vi "Data Readers and Writers NEW.vi"(8 "error in (no error)":errorcluster, 9 "Owning VI Details":T1, 10 "Full Element Name":string[](array[string]), 11 "synchronization":refnum<class "synchronization.lvclass">) -> (0 "error out":errorcluster)   [LabVIEW 2020]
uses:
  synchronization/synchronization.lvclass
  synchronization/synchronization.lvclass/synchronization.ctl
  JKI State Machine API/source/JKI SM/JKI SM.lvclass/JKI SM.ctl
  f42ed989-8671-4cdf-8706-bf1e8fb35ac6.vi
  <vilib>/Utility/error.llb/Clear Errors.vi
  <userlib>/_OpenG.lib/error/error.llb/Filter Error Codes (Array)__ogtk.vi
  <vilib>/regexp/Match Regular Expression.xnode
  <userlib>/_OpenG.lib/comparison/comparison.llb/openg_comparison__ogtk.lvlib
  JKI State Machine API/source/JKI SM/JKI SM.lvclass
  <userlib>/_OpenG.lib/error/error.llb/openg_error.lvlib
  <userlib>/_OpenG.lib/string/string.llb/openg_string.lvlib
  <userlib>/_OpenG.lib/comparison/comparison.llb/I32 Changed__ogtk.vi
  <userlib>/_OpenG.lib/comparison/comparison.llb/Boolean Changed__ogtk.vi
panel:
  in  "Listbox":i32(listbox)
  in  "OK":bool
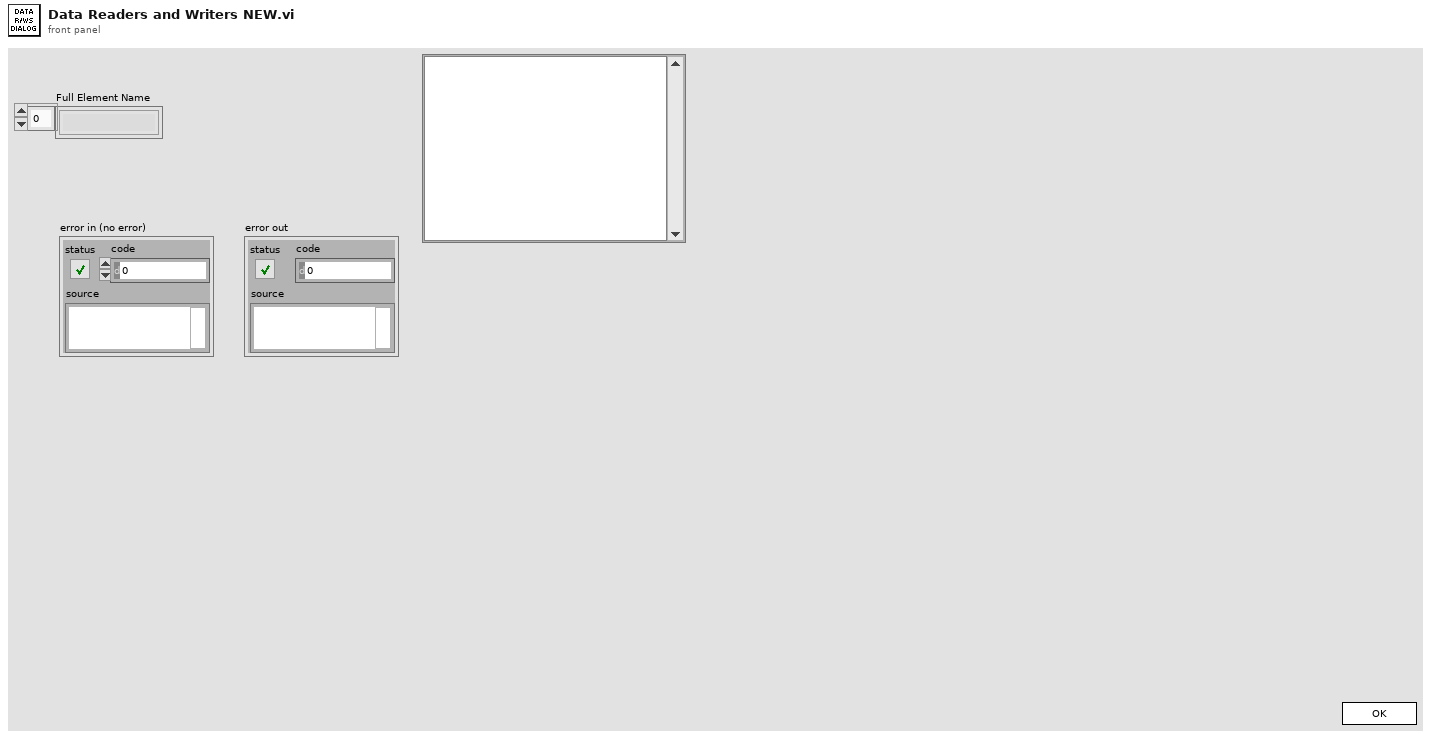
[diagram p1: front panel]
types:
  T1 = cluster{"App.ContextName":string, "VI.Name":string, "Object UID":i32}
  T2 = enum32{"Invalid", "Standard", "Closed", "Hidden", "Minimized", "Maximized"}
  T3 = enum32{"invalid app kind", "Development System", "Run Time System", "Student Edition", "Embedded LabVIEW", "Evaluation", "Custom"}
  T4 = enum32{"Invalid", "Default", "Floating", "Floating/Auto-Hide", "Modal"}
  T5 = cluster{"Core":cluster{"Current VI Reference":refnum<vi>, "Close Panel on Exit?":bool}, "Your Boolean data":bool, "Your string data":string, "Full Element Name":string[], "JKI SM out":refnum<class "JKI SM.lvclass">, "Callers":cluster{"(Un)Bundler":refnum<vi>, "Structure":string, "Frame Name":string}[], "GObject":refnum<vi>}
  T6 = cluster{"(Un)Bundler":refnum<vi>, "Structure":string, "Frame Name":string}[]
  T7 = cluster{"GObject":refnum<vi>, "Structure":string, "Frame Name":string}
  T8 = cluster{"(Un)Bundler":refnum<vi>, "Structure":string, "Frame Name":string}
  T9 = typedef "LVPoint32TypeDef.ctl" = cluster{"Horizontal":i32, "Vertical":i32}
  T10 = cluster{"Shift":bool, "Ctrl":bool, "Alt":bool, "Cmd":bool, "Opt":bool}
  T11 = cluster{"StringConstant":refnum<vi>, "Structure":string, "Frame Name":string, "State Call":string, "UID":dbl}[]
  T12 = cluster{"Current VI Reference":refnum<vi>, "Close Panel on Exit?":bool}
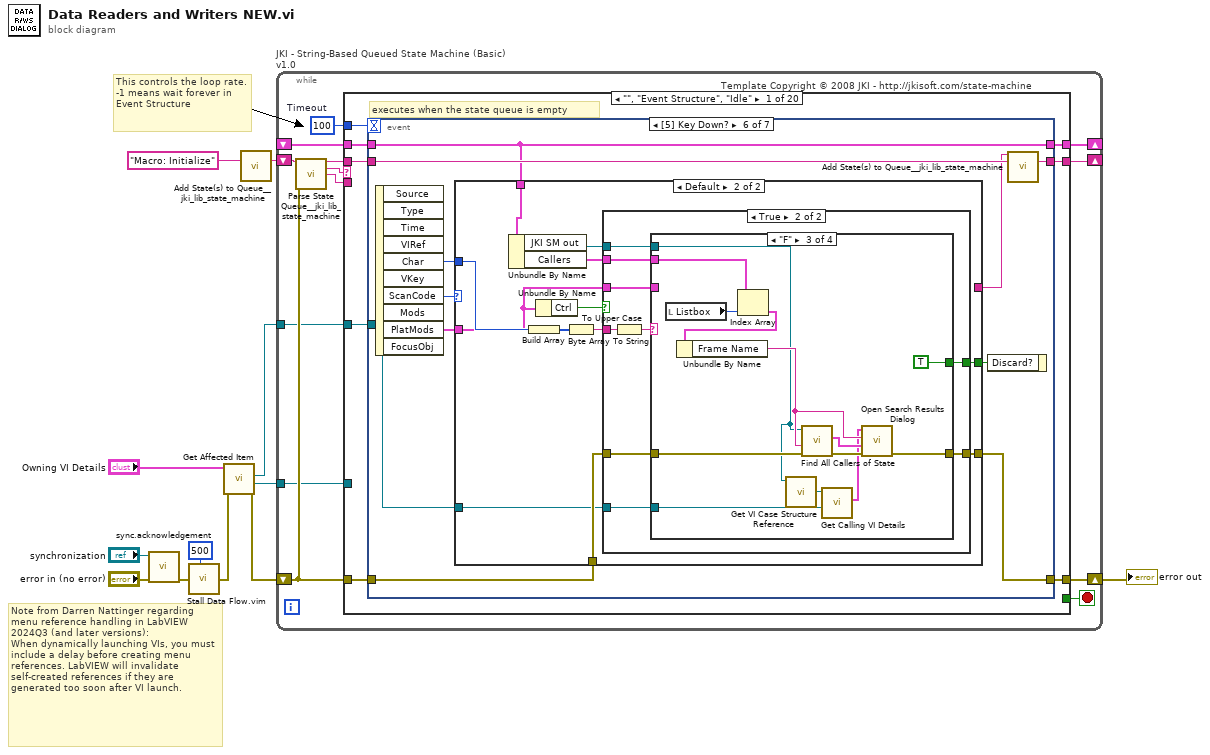
[diagram p0: block diagram]
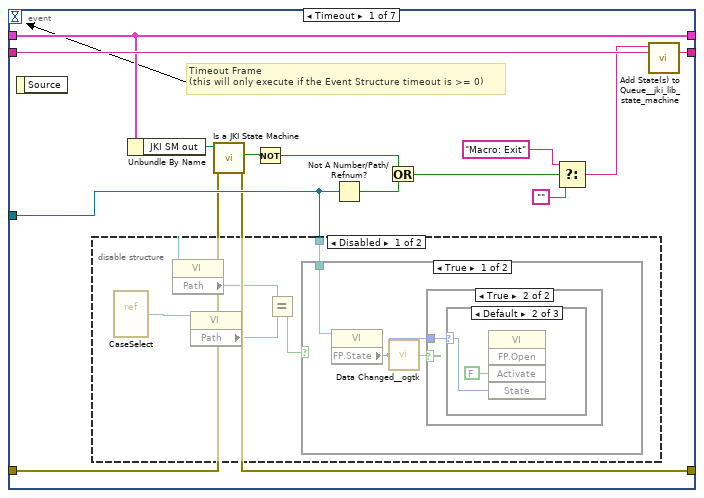
[diagram p2: hidden frame]
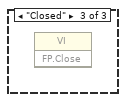
[diagram p5: hidden frame]
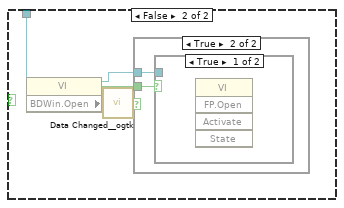
[diagram p6: hidden frame]
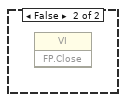
[diagram p8: hidden frame]
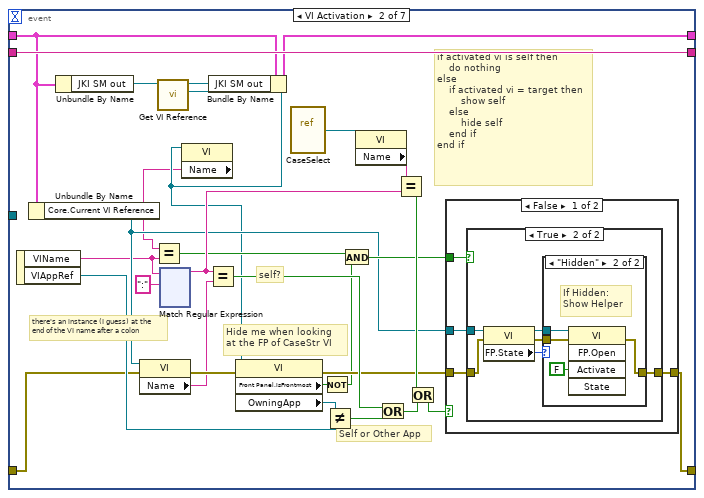
[diagram p10: hidden frame]
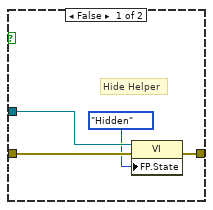
[diagram p11: hidden frame]
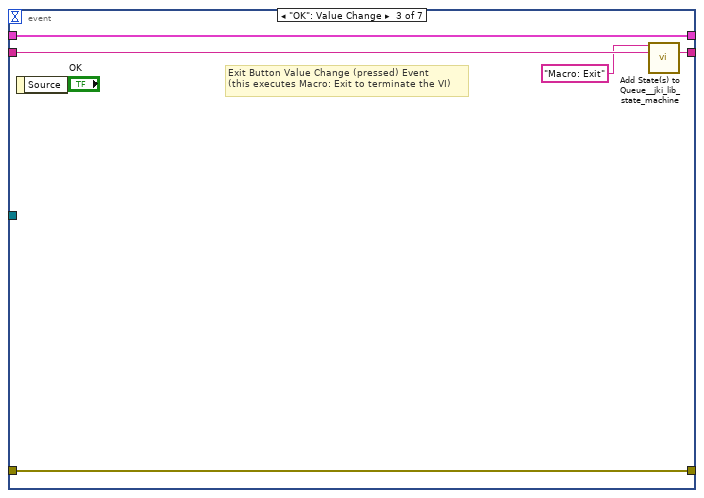
[diagram p14: hidden frame]
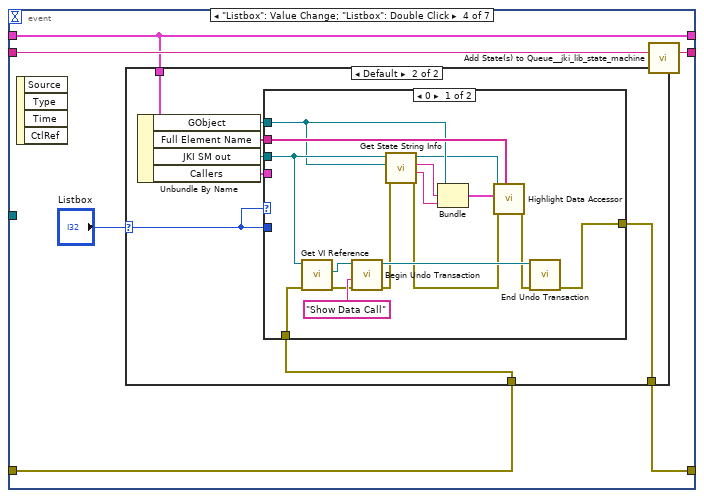
[diagram p15: hidden frame]
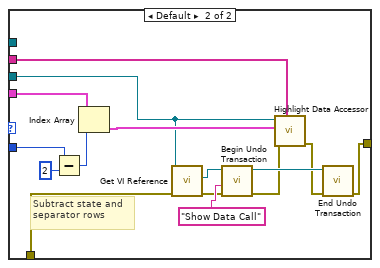
[diagram p17: hidden frame]
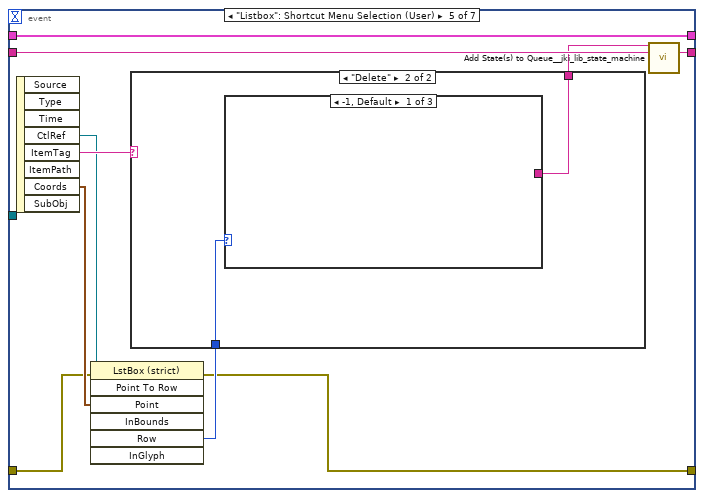
[diagram p18: hidden frame]
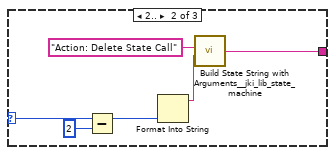
[diagram p20: hidden frame]
diagram:
  # "Note from Darren Nattinger regarding menu reference handling in LabVIEW 2024Q3 (and later versions):\nWhen dynamically launching VIs, you must include a delay before creating menu references. LabVIEW will invalidate self-created references if they are generated too soon after VI launch."
  # "This controls the loop rate. -1 means wait forever in Event Structure"
  n1 = call "sync.acknowledgement.vi"("error in (no error)"="error in (no error)", "synchronization"="synchronization") -> ("error out"=w2:errorcluster)  [unwired: 9 in]
  n2 = call "Stall Data Flow.vim"("value in"=w2, "milliseconds to wait"=u32 500) -> ("value out"=w5:errorcluster)  [unwired: 1 out]
  n3 = call "Get Affected Item.vi"("error in (no error)"=w5, "Owning VI Details"="Owning VI Details") -> ("error out"=w6:errorcluster, "GObject"=w9:refnum<vi>, "Owning VI"=w8:refnum<vi>)  [unwired: 6 in, 1 out]
  n4 = call <vilib>:"Add State(s) to Queue__jki_lib_state_machine.vi"("State(s) in (\"\")"="Macro: Initialize") -> ("States Out"=w12:string)  [unwired: 14 in]
  n5 = while "JKI - String-Based Queued State Machine (Basic) v1.0" {
    shift-right: [w18] -> _
    shift-left: _ -> [w17]
    shift-right: [w21] -> w10
    shift-left: w6 -> [w15]
    shift-right: [w20] -> _
    shift-left: w12 -> [w22]
    tunnel: w8 -> [w14]
    tunnel: w9 -> [w13]
    stop <- w19 stop-if-true
    w16 = 100  # Timeout
    # "Template Copyright © 2008 JKI - http://jkisoft.com/state-machine"
    n6 = call <vilib>:"Parse State Queue__jki_lib_state_machine.vi"("State Queue"=w22, "Error In (no error)"=w15) -> ("Remaining States"=w24:string, "Current State"=w25:string, "Arguments"=w23:string)  [unwired: 11 in]
    n7 = case shown="\"\", \"Event Structure\", \"Idle\"" w25 {
      selector: w25 -> [_ _ w388 _ _ _ _ _ _ _ _ _ _ _ _ _ _ _ _ _]
      tunnel: w24 -> [w33 w387 w392 w412 w423 w428 w432 w444 w458 w464 w485 w503 w523 w534 w563 w568 w578 w582 w599 w643]
      tunnel: w23 -> [_ _ _ _ _ _ _ _ _ _ _ _ w518 w528 _ _ _ _ _ _]
      tunnel: w17 -> [w31 w384 w390 w404 w420 w426 w429 _ w455 w461 w483 w497 w521 w530 w560 w566 w575 w579 w595 w641]
      tunnel: [w30 w385 w394 w399 errorcluster {"status"=FALSE, "code"=0, "source"=""} ("error out") w425 w430 w433 w451 w462 w465 w494 w519 w531 w561 w564 w576 w580 w587 w626] -> w21
      tunnel: w15 -> [w29 w385 w393 w400 w418 w425 w430 w434 w446 w462 w465 w495 w520 w532 w561 w564 w576 w580 w596 w625]
      tunnel: [w32 w386 w391 w411 w422 w427 w431 w443 w457 w463 w484 w502 w522 w533 w562 w567 w577 w581 w598 w642] -> w20
      tunnel: [_ _ _ _ _ TRUE _ _ _ _ _ _ _ _ _ _ _ _ _ _] -> w19
      tunnel: [w28 w384 w390 w410 w420 w426 w429 w442 w455 w461 w483 w497 w521 w530 w560 w566 w575 w579 w584 w640] -> w18
      tunnel: w16 -> [w27 _ _ _ _ _ _ _ _ _ _ _ _ _ _ _ _ _ _ _]
      tunnel: w14 -> [w26 _ _ _ _ _ _ _ _ _ _ _ _ _ _ _ _ _ _ _]
      tunnel: w13 -> [_ _ _ _ _ _ _ w436 _ _ _ _ _ _ _ _ _ _ _ _]
      frame "", "Event Structure", "Idle" {
        # "executes when the state queue is empty"
        n8 = event shown="[5] Key Down?" {
          selector: _ -> [_ _ _ _ _ _ _]
          dyn-events: _ -> [_ _ _ _ _ _ _]
          timeout: w27 -> [_ _ _ _ _ _ _]
          tunnel: w33 -> [w47 w93 w229 w235 w285 w306 w383]
          tunnel: [w46 w93 w228 w234 w284 w305 w382] -> w32
          tunnel: w31 -> [w41 w67 w226 w233 w277 w304 w380]
          tunnel: [w36 w68 w227 w231 w276 w299 w381] -> w30
          tunnel: w29 -> [w37 w69 w227 w232 w279 w300 w381]
          tunnel: [w41 w66 w226 w233 w277 w304 w380] -> w28
          tunnel: w26 -> [w42 _ _ _ _ w296 _]
          event Timeout {
            # "Timeout Frame\n(this will only execute if the Event Structure timeout is >= 0)"
            n9 = event-data() -> ()  [unwired: 1 in, 1 out]
            n10 = disable-structure shown="Disabled" {
              disable-tunnel: w42 -> [w48 _]
              frame Disabled {
                n11 = vi-ref "CaseSelect.vi"() -> (w50:refnum<vi>)
                n12 = property class="VI"(reference=w48) -> ("Path"=w49:path)  [unwired: 1 in, 2 out]
                n13 = property class="VI"(reference=w50) -> ("Path"=w52:path)  [unwired: 1 in, 2 out]
                n14 = Equal?(x=w49, y=w52) -> (x = y?=w51:bool)
                n15 = case shown="True" w51 {
                  tunnel: w48 -> [w53 w60]
                  frame True {
                    n16 = property class="VI"(reference=w53) -> ("FP.State"=w54:T2)  [unwired: 1 in, 2 out]
                    n17 = call-poly <userlib>:"Data Changed__ogtk.vi"("I32"=w54) -> ("Changed"=w55:bool)
                    n18 = case shown="True" w55 {
                      tunnel: w54 -> [_ w56]
                      frame False {
                      }
                      frame True {
                        n19 = case shown="Default" w56 {
                          selector: w56 -> [_ w57 _]
                          frame "Invalid" {
                          }
                          frame Default {
                            n20 = invoke class="VI" method="FP.Open"("Activate"=FALSE ("Activate?"), "State"=w57) -> ()  [unwired: 3 in, 5 out]
                          }
                          frame "Closed" {
                            n21 = invoke class="VI" method="FP.Close"() -> ()  [unwired: 3 in, 3 out]
                          }
                        }
                      }
                    }
                  }
                  frame False {
                    n22 = property class="VI"(reference=w60) -> (reference out=w59:refnum<vi>, "BDWin.Open"=w61:bool)  [unwired: 1 in, 1 out]
                    n23 = call-poly <userlib>:"Data Changed__ogtk.vi"("Boolean"=w61) -> ("Changed"=w62:bool)
                    n24 = case shown="True" w62 {
                      tunnel: w61 -> [_ w64]
                      tunnel: w59 -> [_ w63]
                      frame False {
                      }
                      frame True {
                        n25 = case shown="True" w64 {
                          tunnel: w63 -> [_ _]
                          frame True {
                            n26 = invoke class="VI" method="FP.Open"() -> ()  [unwired: 5 in, 5 out]
                          }
                          frame False {
                            n27 = invoke class="VI" method="FP.Close"() -> ()  [unwired: 3 in, 3 out]
                          }
                        }
                      }
                    }
                  }
                }
              }
              frame Enabled {
              }
            }
            n28 = Unbundle By Name(w41) -> ("JKI SM out"=w40:refnum<class "JKI SM.lvclass">)
            n29 = call "Is a JKI State Machine.vi"("error in (no error)"=w37, "JKI SM in"=w40) -> ("error out"=w36:errorcluster, "Is a JKI State Machine"=w39:bool)  [unwired: 7 in, 1 out]
            n30 = Not(x=w39) -> (.not. x?=w38:bool)
            n31 = Not A Number/Path/Refnum?(number/path/refnum=w42) -> (NaN/Path/Refnum?=w35:bool)
            n32 = Or(x=w38, y=w35) -> (x .or. y?=w34:bool)
            n33 = Select(t="Macro: Exit", s=w34, f="") -> (s? t:f=w43:string)
            n34 = call <vilib>:"Add State(s) to Queue__jki_lib_state_machine.vi"("State(s) in Front (\"\")"=w43, "State(s) in (\"\")"=w47) -> ("States Out"=w46:string)  [unwired: 13 in]
          }
          event VI Activation {
            # "Self or Other App"
            # "self?"
            # "Hide me when looking\nat the FP of CaseStr VI"
            # "there's an instance (I guess) at the\nend of the VI name after a colon"
            # "if activated vi is self then\n    do nothing\nelse\n    if activated vi = target then\n        show self\n    else\n        hide self\n    end if\nend if"
            n35 = event-data() -> ("VIName"=w71:string, "VIAppRef"=w70:refnum<vi>)  [unwired: 1 in]
            n36 = Unbundle By Name(w67) -> ("Core.Current VI Reference"=w78:refnum<vi>)
            n37 = Unbundle By Name(w67) -> ("JKI SM out"=w74:refnum<class "JKI SM.lvclass">)
            n38 = property class="VI"(reference=w78, error in=w69) -> (error out=w82:errorcluster, "Name"=w77:string)  [unwired: 1 out]
            n39 = call "Get VI Reference.vi"("JKI SM in"=w74) -> ("VI"=w73:refnum<vi>, "JKI SM out"=w65:refnum<class "JKI SM.lvclass">)  [unwired: 8 in, 1 out]
            n40 = xnode "Match Regular Expression"("input string"=w71, "regular expression"=":") -> ("before match"=w89:string)  [unwired: 3 in, 5 out]
            n41 = property class="VI"(reference=w73) -> ("Name"=w72:string)  [unwired: 1 in, 2 out]
            n42 = Equal?(x=w72, y=w71) -> (x = y?=w75:bool)
            n43 = Equal?(x=w89, y=w77) -> (x = y?=w86:bool)
            n44 = Bundle By Name(cluster=w67, "JKI SM out"=w65) -> (w66:T5)
            n45 = property class="VI"(reference=w73, error in=w82) -> (error out=w81:errorcluster, "Front Panel.IsFrontmost"=w79:bool, "OwningApp"=w84:refnum<vi>)  [unwired: 1 out]
            n46 = vi-ref "CaseSelect.vi"() -> (w87:refnum<vi>)
            n47 = Not(x=w79) -> (.not. x?=w80:bool)
            n48 = Not Equal?(x=w84, y=w70) -> (x != y?=w85:bool)
            n49 = And(x=w75, y=w80) -> (x .and. y?=w83:bool)
            n50 = property class="VI"(reference=w87) -> ("Name"=w88:string)  [unwired: 1 in, 2 out]
            n51 = Or(x=w86, y=w85) -> (x .or. y?=w91:bool)
            n52 = Equal?(x=w88, y=w89) -> (x = y?=w90:bool)
            n53 = Or(x=w90, y=w91) -> (x .or. y?=w92:bool)
            n54 = case shown="False" w92 {
              tunnel: w81 -> [w97 w113]
              tunnel: [w95 w113] -> w68
              tunnel: w78 -> [w96 _]
              tunnel: w83 -> [w94 _]
              frame False {
                n55 = case shown="True" w94 {
                  tunnel: w97 -> [w101 w106]
                  tunnel: w96 -> [w100 w107]
                  tunnel: [w99 w104] -> w95
                  frame False {
                    # "Hide Helper"
                    n56 = property class="VI"(reference=w100, error in=w101, "FP.State"=T2."Hidden" ("Front Panel Window:State")) -> (error out=w99:errorcluster)  [unwired: 1 out]
                  }
                  frame True {
                    n57 = property class="VI"(reference=w107, error in=w106) -> (reference out=w103:refnum<vi>, error out=w102:errorcluster, "FP.State"=w105:T2)
                    n58 = case shown="\"Hidden\"" w105 {
                      tunnel: [w108 w112] -> w104
                      tunnel: w103 -> [_ w111]
                      tunnel: w102 -> [w108 w110]
                      frame Default {
                      }
                      frame "Hidden" {
                        # "If Hidden:\nShow Helper"
                        n59 = invoke class="VI" method="FP.Open"(reference=w111, error in=w110, "Activate"=FALSE ("Activate?")) -> (error out=w112:errorcluster)  [unwired: 2 in, 4 out]
                      }
                    }
                  }
                }
              }
              frame True {
              }
            }
          }
          event "OK": Value Change {
            # "Exit Button Value Change (pressed) Event\n(this executes Macro: Exit to terminate the VI)"
            n60 = event-data() -> ()  [unwired: 1 in, 1 out]
            n61 = call <vilib>:"Add State(s) to Queue__jki_lib_state_machine.vi"("State(s) in Front (\"\")"="Macro: Exit", "State(s) in (\"\")"=w229) -> ("States Out"=w228:string)  [unwired: 13 in]
          }
          event "Listbox": Value Change; "Listbox": Double Click {
            n62 = event-data() -> ()  [unwired: 1 in, 4 out]
            n63 = case shown="Default" "Listbox" {
              selector: "Listbox" -> [_ w238]
              tunnel: w233 -> [_ w244]
              tunnel: w232 -> [w236 w241]
              tunnel: [w236 w240] -> w231
              frame -1 {
              }
              frame Default {
                n64 = Unbundle By Name(w244) -> ("GObject"=w237:refnum<vi>, "Full Element Name"=w239:string[], "JKI SM out"=w242:refnum<class "JKI SM.lvclass">, "Callers"=w243:T6)
                n65 = case shown="0" w238 {
                  tunnel: w243 -> [_ w275]
                  tunnel: w242 -> [w258 w266]
                  tunnel: w241 -> [w259 w262]
                  tunnel: w238 -> [_ w271]
                  tunnel: [w257 w263] -> w240
                  tunnel: w239 -> [w260 w273]
                  tunnel: w237 -> [w256 _]
                  frame 0 {
                    n66 = call "Get VI Reference.vi"("error in (no error)"=w259, "JKI SM in"=w258) -> ("error out"=w254:errorcluster, "VI"=w253:refnum<vi>)  [unwired: 7 in, 1 out]
                    n67 = call "Begin Undo Transaction.vi"("error in (no error)"=w254, "Action"="Show Data Call", "VI in"=w253) -> ("error out"=w246:errorcluster, "VI out"=w252:refnum<vi>)  [unwired: 7 in]
                    n68 = call "Get State String Info.vi"("error in (no error)"=w246, "GObj Refnum in"=w256, "JKI SM in"=w258) -> ("error out"=w245:errorcluster, "Frame Name"=w249:string, "Structure"=w250:string, "JKI SM out"=w251:refnum<class "JKI SM.lvclass">)  [unwired: 5 in]
                    n69 = Bundle("GObject"=w256, "Structure"=w250, "Frame Name"=w249) -> (w248:T7)  [unwired: 1 in]
                    n70 = call "Highlight Data Accessor.vi"("Full Element Name"=w260, "error in (no error)"=w245, "Cluster"=w248, "JKI SM in"=w251) -> ("error out"=w247:errorcluster)  [unwired: 6 in, 1 out]
                    n71 = call "End Undo Transaction.vi"("error in (no error)"=w247, "VI in"=w252) -> ("error out"=w257:errorcluster)  [unwired: 8 in, 1 out]
                  }
                  frame Default {
                    # "Subtract state and separator rows"
                    n72 = Subtract(x=w271, y=2) -> (x-y=w270:i32)
                    n73 = Index Array(array=w275, index=w270) -> (element=w274:T8)
                    n74 = call "Get VI Reference.vi"("error in (no error)"=w262, "JKI SM in"=w266) -> ("error out"=w268:errorcluster, "VI"=w267:refnum<vi>)  [unwired: 7 in, 1 out]
                    n75 = call "Begin Undo Transaction.vi"("error in (no error)"=w268, "Action"="Show Data Call", "VI in"=w267) -> ("error out"=w261:errorcluster, "VI out"=w265:refnum<vi>)  [unwired: 7 in]
                    n76 = call "Highlight Data Accessor.vi"("Full Element Name"=w273, "error in (no error)"=w261, "Cluster"=w274, "JKI SM in"=w266) -> ("error out"=w264:errorcluster)  [unwired: 6 in, 1 out]
                    n77 = call "End Undo Transaction.vi"("error in (no error)"=w264, "VI in"=w265) -> ("error out"=w263:errorcluster)  [unwired: 8 in, 1 out]
                  }
                }
              }
            }
            n78 = call <vilib>:"Add State(s) to Queue__jki_lib_state_machine.vi"("State(s) in (\"\")"=w235) -> ("States Out"=w234:string)  [unwired: 14 in]
          }
          event "Listbox": Shortcut Menu Selection (User) {
            n79 = event-data() -> ("CtlRef"=w282:refnum<vi>, "ItemTag"=w283:string, "Coords"=w281:T9)  [unwired: 1 in, 5 out]
            n80 = invoke class="LstBox (strict)" method="Point To Row"(reference=w282, error in=w279, "Point"=w281) -> (error out=w276:errorcluster, "Row"=w280:i32)  [unwired: 4 in, 5 out]
            n81 = case shown="\"Delete\"" w283 {
              tunnel: w280 -> [_ w287]
              tunnel: [_ w286] -> w278
              frame Default {
              }
              frame "Delete" {
                n82 = case shown="-1, Default" w287 {
                  selector: w287 -> [_ w290 _]
                  tunnel: [_ w291 w294] -> w286
                  frame -1, Default {
                  }
                  frame 2.. {
                    n83 = Subtract(x=w290, y=2) -> (x-y=w289:i32)
                    n84 = Format Into String(w289) -> (resulting string=w292:string)  [unwired: 3 in, 1 out]
                    n85 = call <vilib>:"Build State String with Arguments__jki_lib_state_machine.vi"("Arguments (\"\")"=w292, "State"="Action: Delete State Call") -> ("State with Arguments"=w291:string)  [unwired: 4 in]
                  }
                  frame 0 {
                    n86 = call <vilib>:"Build State String with Arguments__jki_lib_state_machine.vi"("State"="Action: Delete State") -> ("State with Arguments"=w294:string)  [unwired: 5 in]
                  }
                }
              }
            }
            n87 = call <vilib>:"Add State(s) to Queue__jki_lib_state_machine.vi"("State(s) in Front (\"\")"=w278, "State(s) in (\"\")"=w285) -> ("States Out"=w284:string)  [unwired: 13 in]
          }
          event Key Down? {
            n88 = event-data() -> ("Char"=w303:i16, "ScanCode"=w298:i16, "PlatMods"=w302:T10)  [unwired: 1 in, 7 out]
            n89 = case shown="Default" w298 {
              tunnel: w304 -> [_ w325]
              tunnel: w303 -> [_ w323]
              tunnel: w302 -> [_ w320]
              tunnel: [_ w318] -> w301
              tunnel: w300 -> [w308 w316]
              tunnel: [w308 w315] -> w299
              tunnel: [w307 _] -> w297
              tunnel: w296 -> [_ w314]
              frame 83 {
                n90 = local read "Listbox"() -> (w309:i32)
                n91 = case shown="Default" w309 {
                  selector: w309 -> [_ w310]
                  tunnel: [_ w311] -> w307
                  frame -1 {
                  }
                  frame Default {
                    n92 = Format Into String(w310) -> (resulting string=w312:string)  [unwired: 3 in, 1 out]
                    n93 = call <vilib>:"Build State String with Arguments__jki_lib_state_machine.vi"("Arguments (\"\")"=w312, "State"="Action: Delete State Call") -> ("State with Arguments"=w311:string)  [unwired: 4 in]
                  }
                }
              }
              frame Default {
                n94 = Unbundle By Name(w325) -> ("JKI SM out"=w317:refnum<class "JKI SM.lvclass">, "Callers"=w324:T6)
                n95 = Build Array(w323) -> (w322:i16[])
                n96 = Unbundle By Name(w320) -> ("Ctrl"=w319:bool)
                n97 = Byte Array To String(unsigned byte array=w322) -> (string=w321:string)
                n98 = case shown="True" w319 {
                  tunnel: w324 -> [_ w335]
                  tunnel: w321 -> [_ w334]
                  tunnel: w320 -> [_ w333]
                  tunnel: [_ w332] -> w318
                  tunnel: w317 -> [_ w330]
                  tunnel: [w326 w329] -> w315
                  tunnel: w316 -> [w326 w328]
                  tunnel: w314 -> [_ w327]
                  frame False {
                  }
                  frame True {
                    n99 = To Upper Case(1:w334) -> (0:w331:string)
                    n100 = case shown="\"F\"" w331 {
                      tunnel: w335 -> [_ w350 w361 _]
                      tunnel: w333 -> [_ w345 _ w370]
                      tunnel: [_ TRUE TRUE TRUE] -> w332
                      tunnel: w330 -> [_ _ w354 w367]
                      tunnel: [w336 w343 w355 w364] -> w329
                      tunnel: w328 -> [w336 w343 w356 w368]
                      tunnel: w327 -> [_ _ w351 _]
                      frame Default {
                      }
                      frame "G" {
                        w338 = 2 ("y")
                        n101 = local read "Listbox"() -> (w340:i32)
                        n102 = Unbundle By Name(w345) -> ("Shift"=w346:bool)
                        n103 = Array Size(array=w350) -> (size(s)=w337:i32)
                        n104 = Subtract(x=w340, y=w338) -> (x-y=w339:i32)
                        n105 = Decrement(x=w339) -> (x-1=w348:i32)
                        n106 = Increment(x=w339) -> (x+1=w349:i32)
                        n107 = Select(t=w348, s=w346, f=w349) -> (s? t:f=w347:i32)
                        n108 = Quotient & Remainder(x=w347, y=w337) -> (x-y*floor(x/y)=w342:i32)  [unwired: 1 out]
                        n109 = Add(x=w342, y=w338) -> (x+y=w341:i32)
                        n110 = property on="Listbox" class="LstBox (strict)"("Val(Sgnl)"=w341) -> ()  [unwired: 2 in, 2 out]
                      }
                      frame "F" {
                        n111 = local read "Listbox"() -> (w362:i32)
                        n112 = Index Array(array=w361, index=w362) -> (element=w360:T8)
                        n113 = Unbundle By Name(w360) -> ("Frame Name"=w357:string)
                        n114 = call "Get VI Case Structure Reference.vi"("JKI SM in"=w354) -> ("Case Structure ref"=w353:refnum<vi>)  [unwired: 8 in, 2 out]
                        n115 = call "Find All Callers of State.vi"("error in (no error)"=w356, "State Name"=w357, "JKI SM in"=w354) -> ("error out"=w358:errorcluster, "Callers"=w359:T11)  [unwired: 6 in, 1 out]
                        n116 = call "Get Calling VI Details.vi"("User VI Ref"=w351, "Affected Items"=w353) -> ("Calling VI Details"=w352:T1)  [unwired: 9 in]
                        n117 = call "Open Search Results Dialog.vi"("error in (no error)"=w358, "Callers"=w359, "State"=w357, "Calling VI Details"=w352) -> ("error out"=w355:errorcluster)  [unwired: 7 in]
                      }
                      frame "Z" {
                        # "Override Ctrl+Z and Ctrl+Shift+Z\n(Handle them here and target the user's VI)"
                        n118 = call "Get VI Reference.vi"("error in (no error)"=w368, "JKI SM in"=w367) -> ("error out"=w365:errorcluster, "VI"=w366:refnum<vi>)  [unwired: 7 in, 1 out]
                        n119 = Unbundle By Name(w370) -> ("Shift"=w369:bool)
                        n120 = case shown="False" w369 {
                          tunnel: w366 -> [w374 w377]
                          tunnel: w365 -> [w372 w376]
                          tunnel: [w373 w375] -> w364
                          frame False {
                            n121 = invoke class="VI" method="Transaction.Undo"(reference=w374, error in=w372) -> (error out=w373:errorcluster)  [unwired: 1 in, 2 out]
                          }
                          frame True {
                            n122 = invoke class="VI" method="Transaction.Redo"(reference=w377, error in=w376) -> (error out=w375:errorcluster)  [unwired: 1 in, 2 out]
                          }
                        }
                      }
                    }
                  }
                }
              }
            }
            n123 = event-data("Discard?"=w301) -> ()  [unwired: 1 in, 1 out]
            n124 = call <vilib>:"Add State(s) to Queue__jki_lib_state_machine.vi"("State(s) in Front (\"\")"=w297, "State(s) in (\"\")"=w306) -> ("States Out"=w305:string)  [unwired: 13 in]
          }
          event Panel Close? {
            # "Discard the event because we'll close the front panel ourselves in Macro: Exit"
            # "Close Panel button (pressed) Event\n(this executes Macro: Exit to terminate the VI)"
            n125 = event-data() -> ()  [unwired: 1 in, 1 out]
            n126 = event-data("Discard?"=TRUE) -> ()  [unwired: 1 in, 1 out]
            n127 = call <vilib>:"Add State(s) to Queue__jki_lib_state_machine.vi"("State(s) in Front (\"\")"="Macro: Exit", "State(s) in (\"\")"=w383) -> ("States Out"=w382:string)  [unwired: 13 in]
          }
        }
      }
      frame "---------- Core ----------" {
        # "Do not put any code in this frame.\n(it is a separator no-op)"
        n128 = call <vilib>:"Add State(s) to Queue__jki_lib_state_machine.vi"("State(s) in (\"\")"=w387) -> ("States Out"=w386:string)  [unwired: 14 in]
      }
      frame Default {
        w397 = 42 items=["No error", "Argument error", "Memory is full", "Out of zone", "End of file", "File already open", "Generic file I/O error", "File not found", "File permission error", "Disk is full", "Duplicate path", "Too many files open", "System feature not enabled", "Resource file not found", "Cannot add resource", "Resource not found", "Image not found", "Image memory error", "Pen does not exist", "Config type invalid", "Config token not found", "Config parse error", "Config memory error", "Bad external code format", "Bad external code offset", "External code not present", "Null window", "Destroy window error", "Null menu", "Print aborted", "Bad print record", "Print driver error", "Windows error during printing", "Memory error during printing", "Print dialog error", "Generic print error", "Invalid device refnum", "Device not found", "Device parameter error", "Device unit error", "Cannot open device", "Device call aborted", "Generic error", "Cancelled by user", "Object ID too low", "Object ID too high", "Object not in heap", "Unknown heap", "Unknown object (invalid DefProc)", "Unknown object (DefProc not in table)", "Message out of range", "Invalid (null) method", "Unknown message", "Manager call not supported", "Bad address", "Network operation in progress", "Network operation timed out", "Connection is busy", "Network attribute not supported", "Network error", "Address in use", "System out of memory", "Connection aborted", "Connection refused", "Not connected", "Already connected", "Connection closed", "Initialization error (interapplication manager)", "Bad occurrence", "Wait on unbound occurrence handler", "Occurrence queue overflow", "Datalog type conflict", "Unused", "Unrecognized type (interapplication manager)", "Memory corrupt", "Failed to make temporary DLL", "Old CIN version", "Drag socket not found", "Failed to load drop-object", "Failed to register OLE object", "Failed to release OLE object", "Format specifier type mismatch", "Unknown format specifier", "Too few format specifiers", "Too many format specifiers", "Scan failed", "Newer CIN version", "Error converting to variant", "Runtime menu error", "Password tampered", "Variant attribute not found", "Incompatible variant data type", "Event data is not available", "Event Store is not present", "Occurrence is not found", "Event Queue is not created", "Event info is not available", "Refnum passed is NULL", "Error retrieving Class GUID", "Error retrieving CoClass GUID", "Error retrieving TypeLib GUID.", "Bad built application magic bytes.", "Specific driver is different from the specific driver associated with the Logical Name.", "There is no session opened to the class driver.", "Max Error", "MAX - Error with config objects", "MAX - Error loading configuration", "MAX - Group not supported"]
        # "Current State"
        # "Do not delete, rename, or modify this frame.\n(this is used to capture unhandled states and typos)"
        # "Handle mistyped state name (developer tool)"
        n129 = Format Into String(format string="Software Exception: Unhandled State \"%s\"." ("message"), error in=w393, w388) -> (resulting string=w396:string, error out=w395:errorcluster)  [unwired: 1 in]
        n130 = call <vilib>:"Error Cluster From Error Code.vi"("show call chain? (False)"=TRUE, "error in (no error)"=w395, "error message (\"\")"=w396, "error code (0)"=w397) -> ("error out"=w394:errorcluster)  [unwired: 5 in]
        n131 = call <vilib>:"Add State(s) to Queue__jki_lib_state_machine.vi"("State(s) in (\"\")"=w392) -> ("States Out"=w391:string)  [unwired: 14 in]
      }
      frame "Initialize Core Data" {
        # "Do not delete, rename, or modify this frame.\n(this is used to determine panel behavior on exit)"
        # "originally closed?"
        # "exe?"
        # "If panel starts closed or is an EXE, then close it when we exit"
        n132 = property class="VI"() -> ("Clone Name"=w402:string)  [unwired: 2 in, 2 out]
        n133 = Open VI Reference(vi path=w402, error in (no error)=w400) -> (vi reference=w401:refnum<vi>, error out=w399:errorcluster)  [unwired: 4 in]
        n134 = property class="VI"() -> ("Front Panel.Open"=w409:bool)  [unwired: 2 in, 2 out]
        n135 = property class="App"() -> ("App.Kind"=w408:T3)  [unwired: 2 in, 2 out]
        n136 = Not(x=w409) -> (.not. x?=w406:bool)
        n137 = Equal?(x=w408, y=T3."Run Time System" ("Application:Kind")) -> (x = y?=w405:bool)
        n138 = Or(x=w406, y=w405) -> (x .or. y?=w403:bool)
        n139 = Bundle By Name(cluster=w404, "Core.Current VI Reference"=w401, "Core.Close Panel on Exit?"=w403) -> (w410:T5)
        n140 = call <vilib>:"Add State(s) to Queue__jki_lib_state_machine.vi"("State(s) in (\"\")"=w412) -> ("States Out"=w411:string)  [unwired: 14 in]
      }
      frame "Error Handler" {
        w419 = i32[] [1026]  # JKI SM VI Invalid Ref
        # "Unhandled Error -- Display it"
        # "Handle any errors here.\nYou can also output any states to clean-up after errors occur"
        # "Clear error"
        n141 = call-poly <userlib>:"Filter Error Codes__ogtk.vi"("Error In"=w418, "Error Codes to Filter"=w419) -> ("Error Out"=w417:errorcluster, "Error Filtered?"=w416:bool)  [unwired: 7 in, 1 out]
        n142 = call <vilib>:"General Error Handler.vi"("error in (no error)"=w417) -> ()  [unwired: 10 in, 5 out]
        n143 = Select(t="Macro: Exit", s=w416, f="") -> (s? t:f=w413:string)
        n144 = call <vilib>:"Add State(s) to Queue__jki_lib_state_machine.vi"("State(s) in Front (\"\")"=w413, "State(s) in (\"\")"=w423) -> ("States Out"=w422:string)  [unwired: 13 in]
      }
      frame "Exit" {
        # "Do not put any code in this frame.\n(No errors that occur here will be handled.)"
        n145 = call <vilib>:"Add State(s) to Queue__jki_lib_state_machine.vi"("State(s) in (\"\")"=w428) -> ("States Out"=w427:string)  [unwired: 14 in]
      }
      frame "---------- Data ----------" {
        # "Do not put any code in this frame.\n(It is a separator no-op. You can make a copy of this frame to create a new Data frame)"
        n146 = call <vilib>:"Add State(s) to Queue__jki_lib_state_machine.vi"("State(s) in (\"\")"=w432) -> ("States Out"=w431:string)  [unwired: 14 in]
      }
      frame "Data: Initialize" {
        w437 = T6 []  # Callers
        w439 = T12 {"Current VI Reference"=refnum, "Close Panel on Exit?"=FALSE}  # Core
        w441 = TRUE  # Your Boolean data
        w440 = ""  # Your string data
        # "do not delete - used by framework"
        # "Expand Bundle to add new data elements to shift register data."
        # "Add new data here."
        # "Data names and types of shift register data are defined by this bundle."
        # "Initialize the shift-register data, here.\n(data names are defined by what you wire into the bundle function)"
        n147 = call "Create (From GObject).vi"("error in (no error)"=w434, "GObject"=w436) -> ("error out"=w433:errorcluster, "JKI SM out"=w435:refnum<class "JKI SM.lvclass">)  [unwired: 6 in, 2 out]
        n148 = Bundle("Core"=w439, "Your Boolean data"=w441, "Your string data"=w440, "Full Element Name"="Full Element Name", "JKI SM out"=w435, "Callers"=w437, "GObject"=w436) -> (w442:T5)  [unwired: 1 in]
        n149 = call <vilib>:"Add State(s) to Queue__jki_lib_state_machine.vi"("State(s) in (\"\")"=w444) -> ("States Out"=w443:string)  [unwired: 14 in]
      }
      frame "Data: Cleanup" {
        # "Ignore Errors\n(e.g. reference already invalid)"
        # "Cleanup any data and references, here.\n(this is called automatically, by the Macro: Exit)"
        n150 = Unbundle By Name(w455) -> ("Core.Current VI Reference"=w456:refnum<vi>, "Callers"=w454:T6, "JKI SM out"=w448:refnum<class "JKI SM.lvclass">)
        n151 = for {
          tunnel: w454 -> [w460] mode=indexing
          tunnel: [w459] -> w453 mode=indexing
          n152 = Unbundle By Name(w460) -> ("(Un)Bundler"=w459:refnum<vi>)
        }
        n153 = Close Reference(reference=w456, error in (no error)=w446) -> (error out=w452:errorcluster)
        n154 = Close Reference(reference=w453, error in (no error)=w446) -> (error out=w450:errorcluster)
        n155 = call "Destroy.vi"("error in (no error)"=w446, "JKI SM in"=w448) -> ("error out"=w447:errorcluster)  [unwired: 9 in]
        n156 = call <userlib>:"Clear All Errors__ogtk.vi"("Upsteam Error (optional)"=w446, "Error In"=w447) -> ("Error Out"=w445:errorcluster)  [unwired: 2 in]
        n157 = call <userlib>:"Clear All Errors__ogtk.vi"("Upsteam Error (optional)"=w446, "Error In"=w450) -> ("Error Out"=w449:errorcluster)  [unwired: 2 in]
        n158 = Merge Errors(w452, w449, w445) -> (w451:errorcluster)
        n159 = call <vilib>:"Add State(s) to Queue__jki_lib_state_machine.vi"("State(s) in (\"\")"=w458) -> ("States Out"=w457:string)  [unwired: 14 in]
      }
      frame "---------- UI ----------" {
        # "Do not put any code in this frame.\n(It is a separator no-op. You can make a copy of this frame to create a new UI frame)"
        n160 = call <vilib>:"Add State(s) to Queue__jki_lib_state_machine.vi"("State(s) in (\"\")"=w464) -> ("States Out"=w463:string)  [unwired: 14 in]
      }
      frame "UI: Initialize" {
        # "Initialize the User Interface, here.\n(this is called automatically, by the Macro: Init)"
        n161 = Unbundle By Name(w483) -> ("Core.Current VI Reference"=w482:refnum<vi>, "Full Element Name"=w470:string[], "Callers"=w466:T6)
        n162 = for {
          tunnel: w466 -> [w493] mode=indexing
          tunnel: [w488] -> w476 mode=indexing if=w487
          tunnel: [w488] -> w467 mode=indexing if=w486
          n163 = Unbundle By Name(w493) -> ("Structure"=w489:string, "Frame Name"=w492:string)
          n164 = Equal?(x="EventStructure" ("Structure"), y=w489) -> (x = y?=w487:bool)
          n165 = Format Into String(format string="%s: %s", w489, w492) -> (resulting string=w488:string)  [unwired: 2 in, 1 out]
          n166 = Not(x=w487) -> (.not. x?=w486:bool)
        }
        n167 = call <userlib>:"1D Array to String__ogtk.vi"("delimiter (Tab)"=".", "Array of Strings"=w470) -> ("delimited string"=w468:string)  [unwired: 9 in]
        n168 = Format Into String(format string="Data Accessors (%s)", w468) -> (resulting string=w480:string)  [unwired: 2 in, 1 out]
        n169 = property class="VI"(reference=w482, "Front Panel.Title"=w480) -> ()  [unwired: 1 in, 2 out]
        n170 = Build Array (concatenate)(w468, "" ("format string"), w476, w467) -> (w477:string[])
        n171 = property on="Listbox" class="LstBox (strict)"("Item Names"=w477, "Value"=-1 ("Listbox")) -> (error out=w475:errorcluster, "Item Symbols"=w474:i32[])  [unwired: 2 in, 1 out]
        n172 = Replace Array Subset(array=w474, new element=-1 ("new element/subarray"), index=1) -> (w473:i32[])
        n173 = property on="Listbox" class="LstBox (strict)"(error in=w475, "Item Symbols"=w473) -> ()  [unwired: 1 in, 2 out]
        n174 = call <vilib>:"Add State(s) to Queue__jki_lib_state_machine.vi"("State(s) in (\"\")"=w485) -> ("States Out"=w484:string)  [unwired: 14 in]
      }
      frame "UI: Pre-Test for 0 or 1 Items" {
        n175 = Unbundle By Name(w497) -> ("JKI SM out"=w498:refnum<class "JKI SM.lvclass">, "Full Element Name"=w500:string[], "Callers"=w499:T6)
        n176 = Array Size(array=w499) -> (size(s)=w501:i32)
        n177 = case shown="1" w501 {
          tunnel: w500 -> [_ w507 w511]
          tunnel: [_ "Macro: Exit" "Macro: Exit"] -> w496
          tunnel: w499 -> [_ _ w516]
          tunnel: w498 -> [_ _ w515]
          tunnel: w495 -> [w504 w505 w513]
          tunnel: [w504 w505 w512] -> w494
          frame Default {
          }
          frame 0 {
            n178 = disable-structure shown="Disabled" {
              disable-tunnel: w507 -> [w510 _]
              frame Disabled {
                n179 = Format Into String(format string="State %s has no callers.", w510) -> (resulting string=w508:string)  [unwired: 2 in, 1 out]
                n180 = One Button Dialog(message=w508) -> ()  [unwired: 1 in, 1 out]
              }
              frame Enabled {
              }
            }
          }
          frame 1 {
            n181 = Index Array(array=w516) -> (element=w514:T8)  [unwired: 1 in]
            n182 = call "Highlight Data Accessor.vi"("Full Element Name"=w511, "error in (no error)"=w513, "Cluster"=w514, "JKI SM in"=w515) -> ("error out"=w512:errorcluster)  [unwired: 6 in, 1 out]
          }
        }
        n183 = call <vilib>:"Add State(s) to Queue__jki_lib_state_machine.vi"("State(s) in Front (\"\")"=w496, "State(s) in (\"\")"=w503) -> ("States Out"=w502:string)  [unwired: 13 in]
      }
      frame "UI: Cursor Set" {
        # "Argument"
        # "Set and Unset Cursor Busy.\n(Usage: \"UI: Cursor Set >> Busy|Idle\")"
        n184 = case shown="\"Idle\", Default" w518 {
          tunnel: w520 -> [w525 w527]
          tunnel: [w524 w526] -> w519
          frame "Idle", Default {
            n185 = call <vilib>:"Unset Busy.vi"("error in (no error)"=w525) -> ("error out"=w524:errorcluster)  [unwired: 10 in]
          }
          frame "Busy" {
            n186 = call <vilib>:"Set Busy.vi"("error in (no error)"=w527) -> ("error out"=w526:errorcluster)  [unwired: 9 in, 1 out]
          }
        }
        n187 = call <vilib>:"Add State(s) to Queue__jki_lib_state_machine.vi"("State(s) in (\"\")"=w523) -> ("States Out"=w522:string)  [unwired: 14 in]
      }
      frame "UI: Front Panel State" {
        # "Argument"
        # "Set Front Panel Open or Closed\n(Usage: \"UI: Front Panel State >> Open|Close\")"
        n188 = Unbundle By Name(w530) -> ("Core.Current VI Reference"=w529:refnum<vi>)
        n189 = case shown="\"Open\", Default" w528 {
          tunnel: w532 -> [w538 w554]
          tunnel: [w540 w555] -> w531
          tunnel: w529 -> [w539 w552]
          frame "Open", Default {
            n190 = property class="VI"(reference=w539, error in=w538) -> (reference out=w536:refnum<vi>, error out=w537:errorcluster, "Front Panel.Open"=w535:bool)
            n191 = case shown="False" w535 {
              tunnel: [w543 w549] -> w540
              tunnel: w537 -> [w546 w549]
              tunnel: w536 -> [w545 _]
              frame False {
                # "Setting Floatin here, instead of VI Properties allows the VI to accept keyboard input immediately after openning. (setting it in VI Properties was causing a bug where it wouldn't receive keyboard input until clicking on the VI)"
                n192 = invoke class="VI" method="FP.Open"(reference=w545, error in=w546, "Activate"=TRUE, "State"=T2."Standard") -> (reference out=w542:refnum<vi>, error out=w544:errorcluster)  [unwired: 1 in, 3 out]
                n193 = property class="VI"(reference=w542, error in=w544, "FP.Behavior"=T4."Floating" ("Front Panel Window:Behavior")) -> (error out=w543:errorcluster)  [unwired: 1 out]
              }
              frame True {
              }
            }
          }
          frame "Close" {
            n194 = property class="VI"(reference=w552, error in=w554) -> (reference out=w551:refnum<vi>, error out=w553:errorcluster, "Front Panel.Open"=w550:bool)
            n195 = case shown="True" w550 {
              tunnel: [w556 w559] -> w555
              tunnel: w553 -> [w556 w558]
              tunnel: w551 -> [_ w557]
              frame False {
              }
              frame True {
                n196 = invoke class="VI" method="FP.Close"(reference=w557, error in=w558) -> (error out=w559:errorcluster)  [unwired: 1 in, 2 out]
              }
            }
          }
        }
        n197 = call <vilib>:"Add State(s) to Queue__jki_lib_state_machine.vi"("State(s) in (\"\")"=w534) -> ("States Out"=w533:string)  [unwired: 14 in]
      }
      frame "---------- Macro ----------" {
        # "Do not put any code in this frame.\n(It is a separator no-op. You can make a copy of this frame to create a new Macro frame)"
        n198 = call <vilib>:"Add State(s) to Queue__jki_lib_state_machine.vi"("State(s) in (\"\")"=w563) -> ("States Out"=w562:string)  [unwired: 14 in]
      }
      frame "Macro: Initialize" {
        w565 = "Data: Initialize\nInitialize Core Data\nAction: Find Callers\nAction: Sort Items\nUI: Pre-Test for 0 or 1 Items\nUI: Initialize\nUI: Front Panel State >> Open"  # Data: Initialize Initialize Core Data Action: Find Callers Action: Sort Items UI: Pre-Test for 0 or 1 Items UI: Initialize UI: Front Panel State >> Open
        # "Initialization Macro\n(This is called once, when the VI starts)"
        n199 = call <vilib>:"Add State(s) to Queue__jki_lib_state_machine.vi"("State(s) in Front (\"\")"=w565, "State(s) in (\"\")"=w568) -> ("States Out"=w567:string)  [unwired: 13 in]
      }
      frame "Macro: Exit" {
        # "Exit Macro\n(This is called once, when the VI exits)"
        n200 = Unbundle By Name(w575) -> ("Core.Close Panel on Exit?"=w574:bool)
        n201 = Select(t="UI: Front Panel State >> Close", s=w574, f="") -> (s? t:f=w571:string)
        n202 = call <vilib>:"Add State(s) to Queue__jki_lib_state_machine.vi"("State(s) in (\"\")"=w571, "State(s) at Back (\"\")"="Data: Cleanup\nExit") -> ("States Out"=w569:string)  [unwired: 13 in]
        n203 = call <vilib>:"Add State(s) to Queue__jki_lib_state_machine.vi"("State(s) in Front (\"\")"=w569, "State(s) in (\"\")"=w578) -> ("States Out"=w577:string)  [unwired: 13 in]
      }
      frame "---------- Action ----------" {
        # "Template Separator\n(You can make a copy of, or modify, this frame)"
        n204 = call <vilib>:"Add State(s) to Queue__jki_lib_state_machine.vi"("State(s) in (\"\")"=w582) -> ("States Out"=w581:string)  [unwired: 14 in]
      }
      frame "Action: Sort Items" {
        # "Your code here.\n(You can make a copy of, or modify, this frame)"
        n205 = Unbundle By Name(w595) -> ("Callers"=w593:T6, "JKI SM out"=w594:refnum<class "JKI SM.lvclass">)
        n206 = call "List All Case Frame Names.vi"("error in (no error)"=w596, "JKI SM in"=w594) -> ("error out"=w588:errorcluster, "Case Structure Frame Names"=w597:string[], "JKI SM out"=w592:refnum<class "JKI SM.lvclass">)  [unwired: 6 in, 1 out]
        n207 = call "Get VI Event Structure Reference.vi"("error in (no error)"=w588, "JKI SM in"=w592) -> ("error out"=w589:errorcluster, "Event Structure ref"=w591:refnum<vi>)  [unwired: 7 in, 1 out]
        n208 = property class="EvntStruct"(reference=w591, error in=w589) -> (error out=w587:errorcluster, "EventSelectors"=w590:string[])  [unwired: 1 out]
        n209 = for {
          tunnel: w593 -> [w602]
          tunnel: [w601] -> w586 mode=concatenating
          tunnel: w590 -> [w600] mode=indexing
          n210 = for {
            tunnel: w602 -> [w604] mode=indexing
            tunnel: w600 -> [w609]
            tunnel: [w604] -> w601 mode=indexing if=w603
            n211 = Unbundle By Name(w604) -> ("Structure"=w608:string, "Frame Name"=w610:string)
            n212 = Equal?(x="EventStructure" ("Structure"), y=w608) -> (x = y?=w606:bool)
            n213 = Equal?(x=w610, y=w609) -> (x = y?=w605:bool)
            n214 = And(x=w606, y=w605) -> (x .and. y?=w603:bool)
          }
        }
        n215 = for {
          tunnel: w597 -> [w612] mode=indexing
          tunnel: w593 -> [w613]
          tunnel: [w611] -> w585 mode=concatenating
          n216 = for {
            tunnel: w613 -> [w615] mode=indexing
            tunnel: w612 -> [w620]
            tunnel: [w615] -> w611 mode=indexing if=w614
            n217 = Unbundle By Name(w615) -> ("Structure"=w619:string, "Frame Name"=w621:string)
            n218 = Equal?(x="CaseStructure" ("Structure"), y=w619) -> (x = y?=w617:bool)
            n219 = Equal?(x=w621, y=w620) -> (x = y?=w616:bool)
            n220 = And(x=w617, y=w616) -> (x .and. y?=w614:bool)
          }
        }
        n221 = Build Array (concatenate)(w586, w585) -> (w583:T6)
        n222 = call <vilib>:"Add State(s) to Queue__jki_lib_state_machine.vi"("State(s) in (\"\")"=w599) -> ("States Out"=w598:string)  [unwired: 14 in]
        n223 = Bundle By Name(cluster=w595, "Callers"=w583) -> (w584:T5)
      }
      frame "Action: Find Callers" {
        w633 = T8 {"(Un)Bundler"=refnum, "Structure"="", "Frame Name"=""}  # Callers
        w628 = T6 []  # Callers
        # "Your code here.\n(You can make a copy of, or modify, this frame)"
        n224 = Unbundle By Name(w641) -> ("JKI SM out"=w622:refnum<class "JKI SM.lvclass">, "Full Element Name"=w624:string[])
        n225 = call "Find All Readers of Data.vi"("error in (no error)"=w625, "Full Element Name"=w624, "JKI SM in"=w622) -> ("error out"=w637:errorcluster, "NamedUnbundlers"=w639:refnum<vi>[], "JKI SM out"=w636:refnum<class "JKI SM.lvclass">)  [unwired: 6 in]
        n226 = call "Find All Writers of Data.vi"("error in (no error)"=w637, "Full Element Name"=w624, "JKI SM in"=w636) -> ("error out"=w634:errorcluster, "InPlaceClusterNode"=w630:refnum<vi>[], "NamedBundlers"=w638:refnum<vi>[], "JKI SM out"=w629:refnum<class "JKI SM.lvclass">)  [unwired: 5 in]
        n227 = Build Array (concatenate)(w639, w638, w630) -> (w635:refnum<vi>[])
        n228 = for {
          tunnel: w635 -> [w647] mode=indexing
          shift-right: [w651] -> w623
          shift-left: w629 -> [w652]
          shift-right: [w649] -> w631
          shift-left: w634 -> [w650]
          tunnel: w633 -> [w648]
          tunnel: [w644] -> w632 mode=indexing
          n229 = call "Get State String Info.vi"("error in (no error)"=w650, "GObj Refnum in"=w647, "JKI SM in"=w652) -> ("error out"=w649:errorcluster, "Frame Name"=w645:string, "Structure"=w646:string, "JKI SM out"=w651:refnum<class "JKI SM.lvclass">)  [unwired: 5 in]
          n230 = Bundle By Name(cluster=w648, "(Un)Bundler"=w647, "Structure"=w646, "Frame Name"=w645) -> (w644:T8)
        }
        n231 = call <vilib>:"Add State(s) to Queue__jki_lib_state_machine.vi"("State(s) in (\"\")"=w643) -> ("States Out"=w642:string)  [unwired: 14 in]
        n232 = Variant To Data(error in=w631, type=w628, Variant=w632) -> (data=w627:T6, error out=w626:errorcluster)
        n233 = Bundle By Name(cluster=w641, "JKI SM out"=w623, "Callers"=w627) -> (w640:T5)
      }
    }
  }
  "error out" <- w10
